vi "FindStateInArray.vi"(9 "TransactionState":string, 10 "AllCaseStates":string[](array[string])) -> (1 "CaseStateOut":string, 2 "index of element":i32, 3 "AllIndexes":i32[](array[numeric]))   [LabVIEW 2020, in "StateReverse.lvclass"]
uses:
  <resource>/Framework/Providers/Open_GDS/UML/StateReverse_class/StateReverse.lvclass
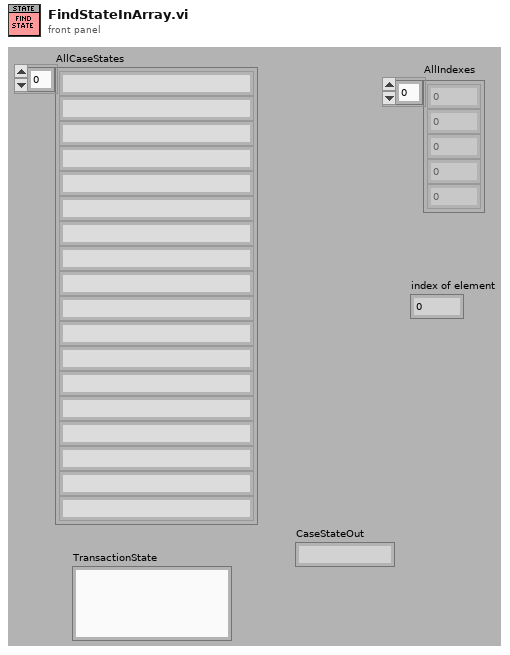
[diagram p1: front panel]
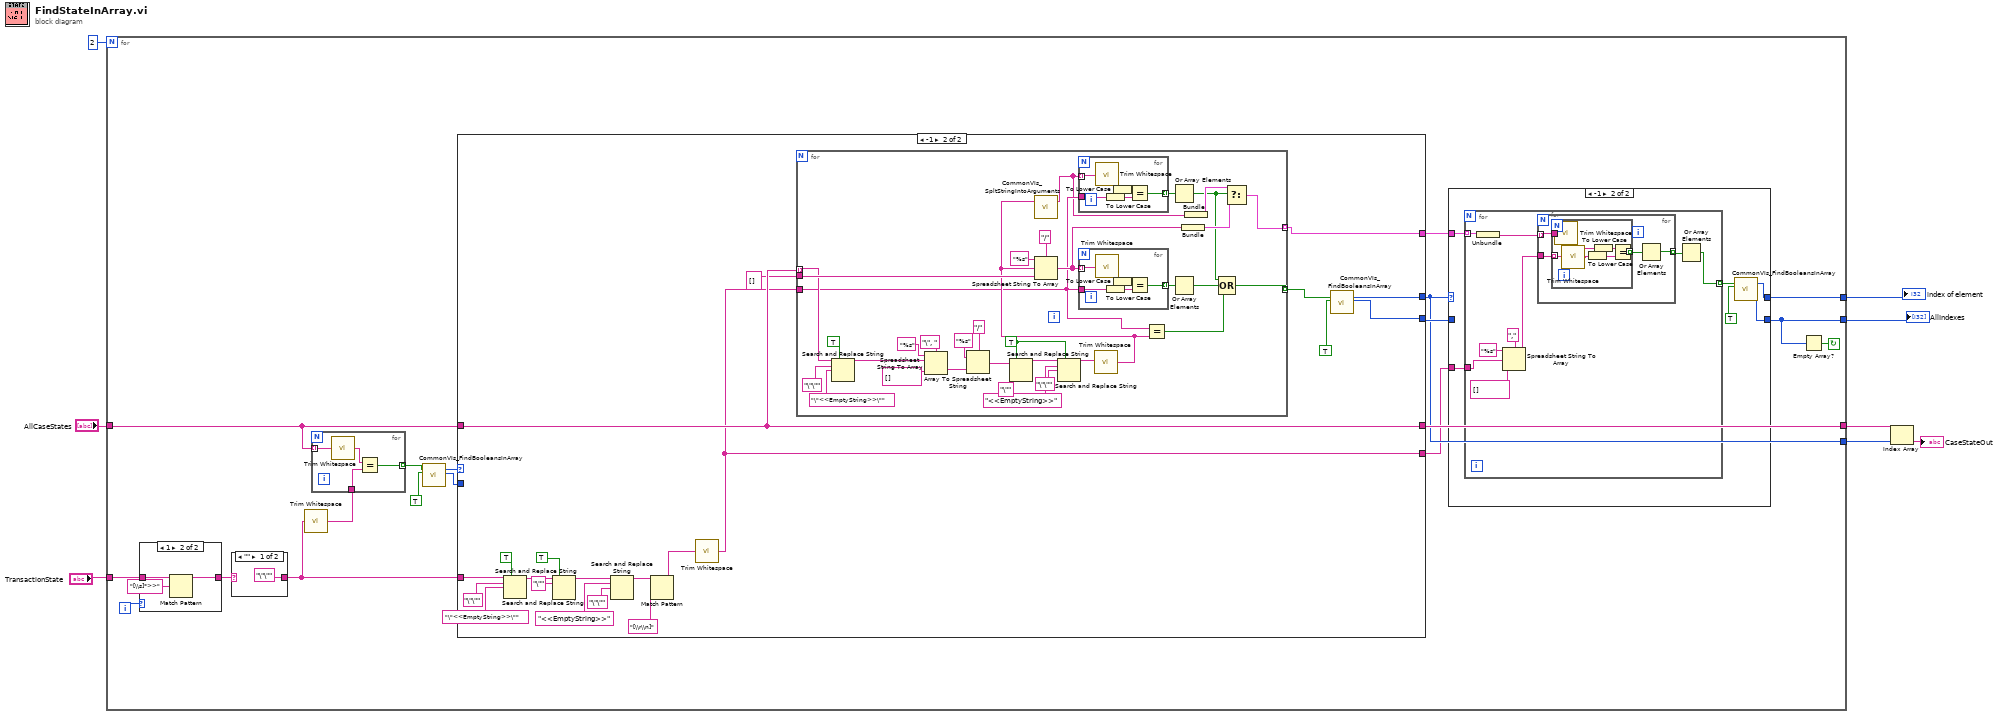
[diagram p0: block diagram]
diagram:
  n1 = for {
    N: 2 -> [_]
    tunnel: "TransactionState" -> [w12]
    tunnel: "AllCaseStates" -> [w25]
    tunnel: [w24] -> w6
    tunnel: [w17] -> w4
    tunnel: [w10] -> w3
    tunnel: [w16] -> w2
    i -> [w13]
    stop <- w9 continue-if-true
    n2 = case shown="1" w13 {
      tunnel: w12 -> [w27 w30]
      tunnel: [w27 w28] -> w11
      frame 0, Default {
      }
      frame 1 {
        n3 = Match Pattern(string=w30, regular expression="[\\s]*>>") -> (before substring=w28:string)  [unwired: 1 in, 3 out]
      }
    }
    n4 = case shown="\"\"" w11 {
      selector: w11 -> [_ w134]
      tunnel: ["\"\"" ("delimiter (Tab)") w134] -> w26
      frame "" {
      }
      frame Default {
      }
    }
    n5 = call <vilib>:"Trim Whitespace.vi"("string"=w26) -> ("trimmed string"=w22:string)  [unwired: 1 in]
    n6 = for {
      tunnel: w25 -> [w132] mode=indexing
      tunnel: w22 -> [w130]
      tunnel: [w129] -> w21 mode=indexing
      n7 = call <vilib>:"Trim Whitespace.vi"("string"=w132) -> ("trimmed string"=w131:string)  [unwired: 1 in]
      n8 = Equal?(x=w131, y=w130) -> (x = y?=w129:bool)
    }
    n9 = call <resource>:"CommonVIs_FindBooleansInArray.vi"("1D array"=w21, "element"=TRUE) -> ("index of element"=w20:i32, "ArrayOfIndexOfElement"=w19:i32[])  [unwired: 16 out]
    n10 = case shown="-1" w20 {
      selector: w20 -> [w60 _]
      tunnel: [w60 w72] -> w17
      tunnel: [w59 w71] -> w18
      tunnel: w26 -> [_ w67]
      tunnel: w25 -> [w61 w66]
      tunnel: [w61 w66] -> w24
      tunnel: w19 -> [w59 _]
      tunnel: [_ w63] -> w15
      tunnel: [_ w62] -> w14
      frame 0, Default {
      }
      frame -1 {
        n11 = Search and Replace String(replace all?=TRUE ("replace all? (F)"), input string=w67, search string="\"\"" ("delimiter (Tab)"), replace string="\"<<EmptyString>>\"" ("delimiter (Tab)")) -> (result string=w77:string)  [unwired: 4 in, 3 out]
        n12 = Search and Replace String(replace all?=TRUE ("replace all? (F)"), input string=w77, search string="\"") -> (result string=w75:string)  [unwired: 5 in, 3 out]
        n13 = Search and Replace String(input string=w75, search string="<<EmptyString>>" ("delimiter (Tab)"), replace string="\"\"" ("delimiter (Tab)")) -> (result string=w70:string)  [unwired: 5 in, 3 out]
        n14 = Match Pattern(string=w70, regular expression="[\\r\\n]") -> (before substring=w68:string)  [unwired: 1 in, 3 out]
        n15 = call <vilib>:"Trim Whitespace.vi"("string"=w68) -> ("trimmed string"=w62:string)  [unwired: 1 in]
        n16 = for {
          tunnel: w66 -> [w94] mode=indexing
          tunnel: [w92] -> w64 mode=indexing
          tunnel: string[] [] -> [w115]
          tunnel: w62 -> [w88]
          tunnel: [w84] -> w63 mode=indexing
          w99 = TRUE ("replace all? (F)")
          n17 = Search and Replace String(replace all?=TRUE ("replace all? (F)"), input string=w94, search string="\"\"" ("delimiter (Tab)"), replace string="\"<<EmptyString>>\"" ("delimiter (Tab)")) -> (result string=w102:string)  [unwired: 1 in, 6 out]
          n18 = Spreadsheet String To Array(delimiter (Tab)="\", ", format string="%s", spreadsheet string=w102, array type (2D Dbl)=string[] []) -> (array=w108:string[])
          n19 = Array To Spreadsheet String(delimiter (Tab)="/", array=w108, 3:"%s" ("format string")) -> (spreadsheet string=w105:string)
          n20 = Search and Replace String(replace all?=w99, input string=w105, search string="\"" ("delimiter (Tab)")) -> (result string=w100:string)  [unwired: 1 in, 7 out]
          n21 = Search and Replace String(replace all?=w99, input string=w100, search string="<<EmptyString>>" ("delimiter (Tab)"), replace string="\"\"" ("delimiter (Tab)")) -> (result string=w95:string)  [unwired: 1 in, 6 out]
          n22 = call <vilib>:"Trim Whitespace.vi"("string"=w95) -> ("trimmed string"=w90:string)  [unwired: 1 in]
          n23 = call <resource>:"CommonVIs_SpltStringIntoArguments.vi"("String"=w90) -> ("splittedString"=w87:string[])  [unwired: 17 in, 1 out]
          n24 = Spreadsheet String To Array(delimiter (Tab)="/", format string="%s", spreadsheet string=w90, array type (2D Dbl)=w115) -> (array=w91:string[])
          n25 = for {
            tunnel: w87 -> [w119] mode=indexing
            tunnel: w88 -> [w122]
            tunnel: [w121] -> w89 mode=indexing
            n26 = call <vilib>:"Trim Whitespace.vi"("string"=w119) -> ("trimmed string"=w120:string)  [unwired: 1 in]
            n27 = To Lower Case(string=w122) -> (all lower case string=w117:string)
            n28 = To Lower Case(string=w120) -> (all lower case string=w118:string)
            n29 = Equal?(x=w118, y=w117) -> (x = y?=w121:bool)
          }
          n30 = for {
            tunnel: w91 -> [w125] mode=indexing
            tunnel: w88 -> [w128]
            tunnel: [w127] -> w113 mode=indexing
            n31 = call <vilib>:"Trim Whitespace.vi"("string"=w125) -> ("trimmed string"=w126:string)  [unwired: 1 in]
            n32 = To Lower Case(string=w128) -> (all lower case string=w123:string)
            n33 = To Lower Case(string=w126) -> (all lower case string=w124:string)
            n34 = Equal?(x=w124, y=w123) -> (x = y?=w127:bool)
          }
          n35 = Equal?(x=w88, y=w90) -> (x = y?=w93:bool)
          n36 = Or Array Elements(Boolean array=w89) -> (logical OR=w83:bool)
          n37 = Or Array Elements(Boolean array=w113) -> (logical OR=w112:bool)
          n38 = Bundle(w91) -> (w85:cluster{string[]})  [unwired: 1 in]
          n39 = Bundle("splittedString"=w87) -> (w86:cluster{"splittedString":string[]})  [unwired: 1 in]
          n40 = Compound Arithmetic op=OR(w83, w112, w93) -> (w92:bool)
          n41 = Select(t=w86, s=w83, f=w85) -> (s? t:f=w84:cluster{"splittedString":string[]})
        }
        n42 = call <resource>:"CommonVIs_FindBooleansInArray.vi"("1D array"=w64, "element"=TRUE) -> ("index of element"=w72:i32, "ArrayOfIndexOfElement"=w71:i32[])  [unwired: 16 out]
      }
    }
    n43 = case shown="-1" w17 {
      selector: w17 -> [w32 _]
      tunnel: [w32 w34] -> w16
      tunnel: [w31 w33] -> w10
      tunnel: w18 -> [w31 _]
      tunnel: w15 -> [_ w37]
      tunnel: w14 -> [_ w38]
      frame 0, Default {
      }
      frame -1 {
        n44 = for {
          tunnel: w38 -> [w41]
          tunnel: w37 -> [w45] mode=indexing
          tunnel: [w39] -> w36 mode=indexing
          n45 = Unbundle(w45) -> ("splittedString"=w43:string[])
          n46 = Spreadsheet String To Array(delimiter (Tab)=",", format string="%s", spreadsheet string=w41, array type (2D Dbl)=string[] []) -> (array=w44:string[])
          n47 = for {
            tunnel: w43 -> [w50] mode=indexing
            tunnel: w44 -> [w51]
            tunnel: [w48] -> w42 mode=indexing
            n48 = for {
              tunnel: w51 -> [w53] mode=indexing
              tunnel: [w58] -> w49 mode=indexing
              tunnel: w50 -> [w56]
              n49 = call <vilib>:"Trim Whitespace.vi"("string"=w56) -> ("trimmed string"=w57:string)  [unwired: 1 in]
              n50 = call <vilib>:"Trim Whitespace.vi"("string"=w53) -> ("trimmed string"=w52:string)  [unwired: 1 in]
              n51 = To Lower Case(string=w52) -> (all lower case string=w54:string)
              n52 = To Lower Case(string=w57) -> (all lower case string=w55:string)
              n53 = Equal?(x=w55, y=w54) -> (x = y?=w58:bool)
            }
            n54 = Or Array Elements(Boolean array=w49) -> (logical OR=w48:bool)
          }
          n55 = Or Array Elements(Boolean array=w42) -> (logical OR=w39:bool)
        }
        n56 = call <resource>:"CommonVIs_FindBooleansInArray.vi"("1D array"=w36, "element"=TRUE) -> ("index of element"=w34:i32, "ArrayOfIndexOfElement"=w33:i32[])  [unwired: 16 out]
      }
    }
    n57 = Empty Array?(array=w10) -> (empty?=w9:bool)
  }
  "index of element" <- w2
  "AllIndexes" <- w3
  n58 = Index Array(array=w6, index=w4) -> (element=→"CaseStateOut":string)
